vi "Global_tst_num.vi"() -> ()   [LabVIEW 2020, in "Sgraph_lib_V1.lvlib"]
uses:
  Builds/Sgraph_lib_V1.lvlib
panel:
  in  "num":dbl format="%.2f"
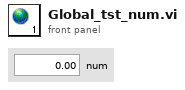
[diagram p1: front panel]
diagram:
